vi "Render.vi"(8 "error in (no error)":errorcluster, 10 "String in":string, 11 "Heading in":refnum<class "Heading.lvclass">) -> (0 "error out":errorcluster, 2 "String out":string, 3 "Heading out":refnum<class "Heading.lvclass">)   [LabVIEW 2021, in "LvMarkdown.lvlib" / "Heading.lvclass"]
uses:
  Heading.lvclass
  C:/GitHub/LvMarkdown/src/LvMarkdown/Markdown.lvclass
  Heading.lvclass/Heading.ctl
  GetHeadingLevel.vi
  GetId.vi
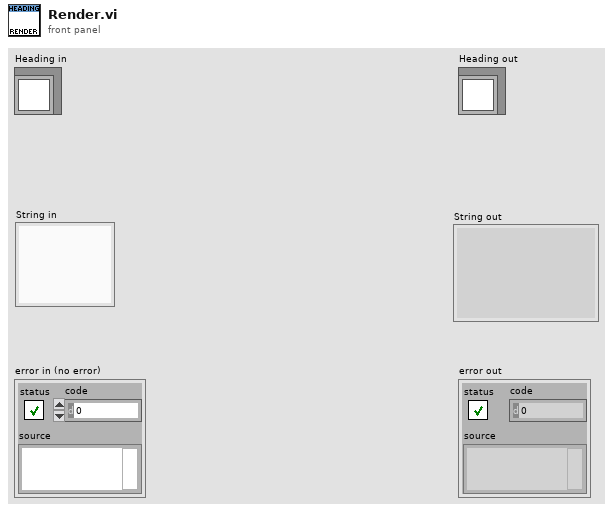
[diagram p1: front panel]
types:
  T1 = enum16{"Level 1", "Level 2", "Level 3", "Level 4", "Level 5", "Level 6"}
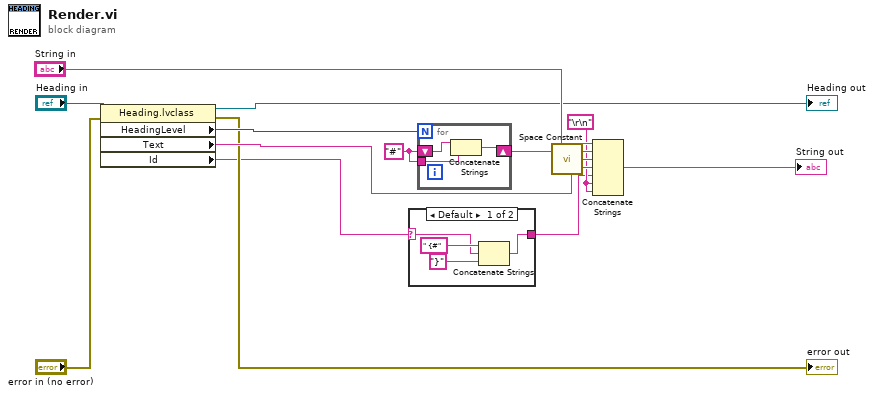
[diagram p0: block diagram]
diagram:
  w5 = "\r\n"
  w12 = "#"
  n1 = property class="Heading.lvclass"(reference="Heading in", error in="error in (no error)") -> (reference out=→"Heading out":refnum<class "Heading.lvclass">, error out=→"error out":errorcluster, "HeadingLevel"=w9:T1, "Text"=w8:string, "Id"=w2:string)
  n2 = case shown="Default" w2 {
    selector: w2 -> [w17 w19]
    tunnel: [w16 w19] -> w1
    frame Default {
      n3 = Concatenate Strings(" {#" ("string"), w17, "}" ("string")) -> (w16:string)
    }
    frame "" {
    }
  }
  n4 = for {
    N: w9 -> [_]
    shift-right: [w22] -> w11
    shift-left: w12 -> [w21]
    tunnel: w12 -> [w20]
    n5 = Concatenate Strings(w21, w20) -> (w22:string)
  }
  n6 = call <vilib>:"Space Constant.vi"() -> ("String"=w10:string)
  n7 = Concatenate Strings("String in", w11, w10, w8, w1, w5, w5) -> (→"String out":string)
